vi "SetApiKeys.vi"(8 "error in (no error)":errorcluster, 10 "ApiKeys":string[](array[string]), 11 "ITool in":refnum<class "ITool.lvclass">) -> (0 "error out":errorcluster, 3 "ITool out":refnum<class "ITool.lvclass">)   [LabVIEW 2017, in "ITool.lvclass"]
uses:
  ITool.lvclass
  ITool.lvclass/ITool.ctl
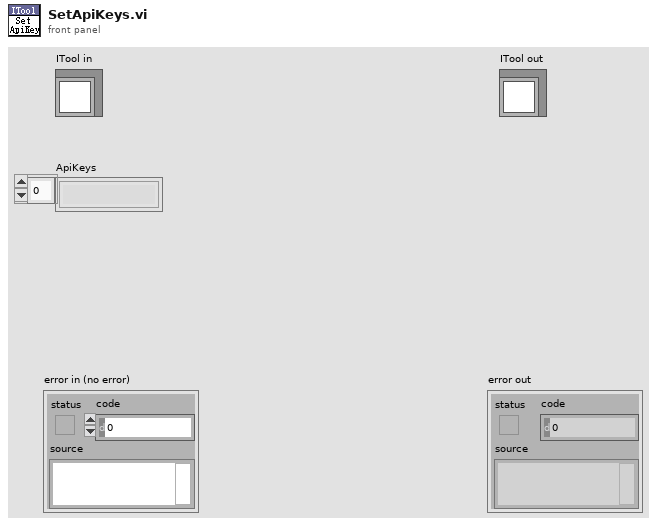
[diagram p1: front panel]
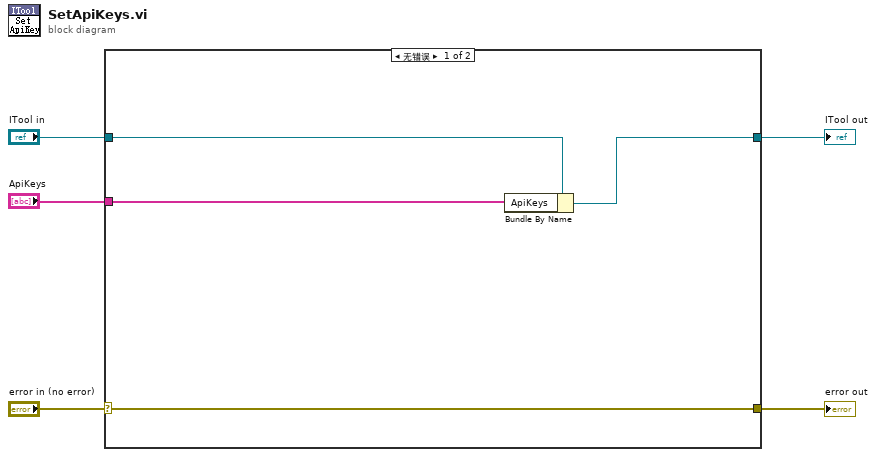
[diagram p0: block diagram]
diagram:
  n1 = case shown="无错误" "error in (no error)" {
    selector: "error in (no error)" -> [w9 w11]
    tunnel: [w9 w11] -> w3
    tunnel: [w6 w10] -> w4
    tunnel: "ITool in" -> [w7 w10]
    tunnel: "ApiKeys" -> [w8 _]
    frame No Error {
      n2 = Bundle By Name(cluster=w7, "ApiKeys"=w8) -> (w6:refnum<class "ITool.lvclass">)
    }
    frame Error {
    }
  }
  "ITool out" <- w4
  "error out" <- w3
